vi "AWS Execute CMD.vi"(8 "error in (no error)":errorcluster, 11 "LV-Data.AWS CLI":refnum<class "LV-Data.AWS CLI.lvclass">) -> (0 "error out":errorcluster, 2 "std out":string, 3 "LV-Data.AWS CLI out":refnum<class "LV-Data.AWS CLI.lvclass">)   [LabVIEW 2019, in "LV-Data.AWS CLI.lvclass"]
uses:
  LV-Data.AWS CLI.lvclass
  <userlib>/_OpenG.lib/string/string.llb/Trim Whitespace (String)__ogtk.vi
panel:
  # "aws --version"
  # "aws s3 ls s3://levylab-data/CF900/"
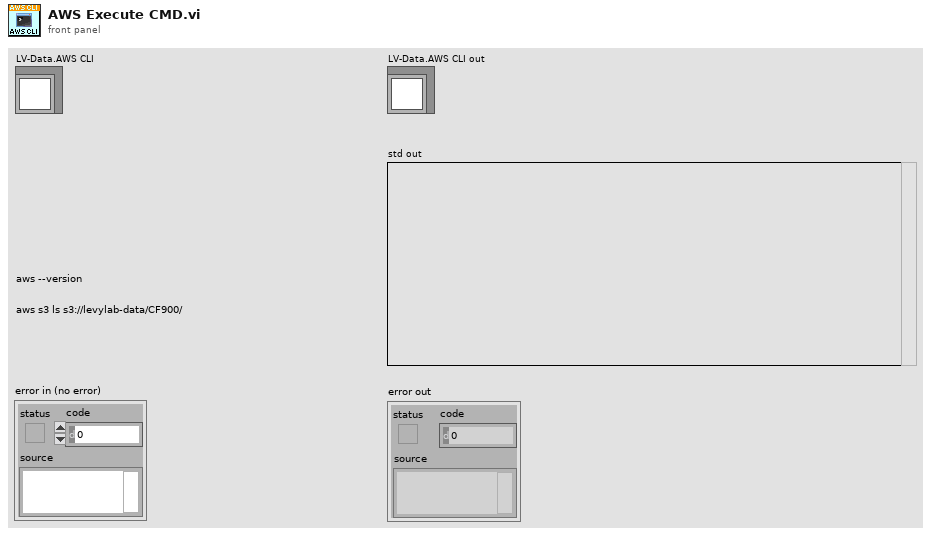
[diagram p1: front panel]
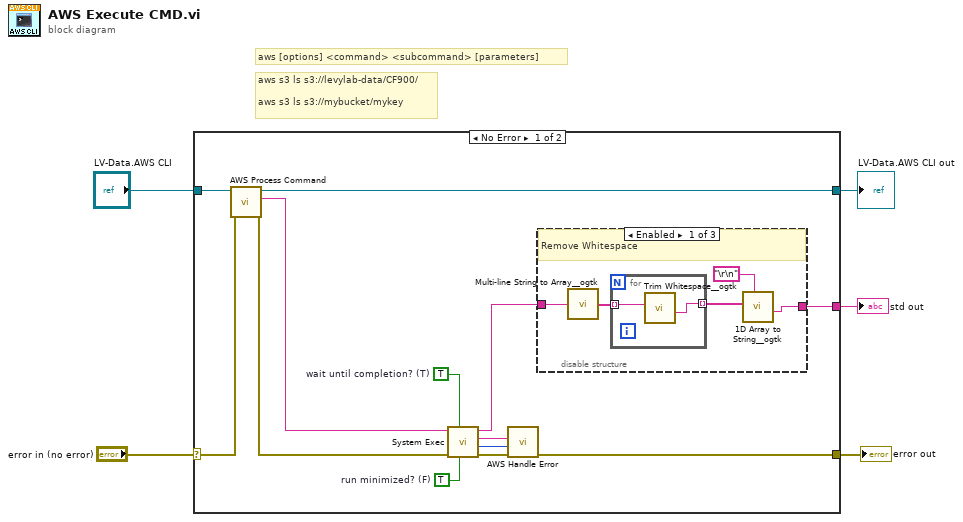
[diagram p0: block diagram]
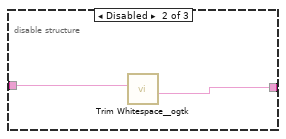
[diagram p2: hidden frame]
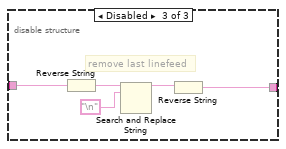
[diagram p3: hidden frame]
diagram:
  # "aws s3 ls s3://levylab-data/CF900/\n\naws s3 ls s3://mybucket/mykey"
  # "aws [options] <command> <subcommand> [parameters]"
  n1 = case shown="No Error" "error in (no error)" {
    selector: "error in (no error)" -> [w13 w34]
    tunnel: [w8 w34] -> w4
    tunnel: [w9 w33] -> w2
    tunnel: "LV-Data.AWS CLI" -> [w10 w33]
    tunnel: [w6 _] -> w1
    frame No Error {
      w17 = TRUE  # wait until completion? (T)
      w18 = TRUE  # run minimized? (F)
      n2 = call "AWS Process Command.vi"("error in"=w13, "LV-Data.AWS CLI"=w10) -> ("error out"=w12:errorcluster, "command line"=w11:string, "LV-Data.AWS CLI out"=w9:refnum<class "LV-Data.AWS CLI.lvclass">)  [unwired: 7 in]
      n3 = call <vilib>:"System Exec.vi"("run minimized? (F)"=w18, "wait until completion? (T)"=w17, "error in (no error)"=w12, "command line"=w11) -> ("error out"=w16:errorcluster, "return code"=w14:i32, "standard error"=w15:string, "standard output"=w7:string)  [unwired: 4 in]
      n4 = call "AWS Handle Error.vi"("error in (no error)"=w16, "return code"=w14, "standard error"=w15) -> ("error out"=w8:errorcluster)  [unwired: 8 in]
      n5 = disable-structure shown="Enabled" {
        disable-tunnel: w7 -> [w23 w27 w29]
        disable-tunnel: [w19 w26 w28] -> w6
        frame Enabled {
          # "Remove Whitespace"
          n6 = call <userlib>:"Multi-line String to Array__ogtk.vi"("string"=w23) -> ("lines"=w22:string[])
          n7 = for {
            tunnel: w22 -> [w25] mode=indexing
            tunnel: [w24] -> w20 mode=indexing
            n8 = call-poly <userlib>:"Trim Whitespace__ogtk.vi"("String in"=w25) -> ("String out"=w24:string)  [unwired: 6 in]
          }
          n9 = call <userlib>:"1D Array to String__ogtk.vi"("delimiter (Tab)"="\r\n", "Array of Strings"=w20) -> ("delimited string"=w19:string)  [unwired: 9 in]
        }
        frame Disabled {
          n10 = call-poly <userlib>:"Trim Whitespace__ogtk.vi"("String in"=w27) -> ("String out"=w26:string)  [unwired: 6 in]
        }
        frame Disabled {
          # "remove last linefeed"
          n11 = Reverse String(1:w29) -> (0:w32:string)
          n12 = Search and Replace String(input string=w32, search string="\n") -> (result string=w31:string)  [unwired: 6 in, 3 out]
          n13 = Reverse String(1:w31) -> (0:w28:string)
        }
      }
    }
    frame Error {
    }
  }
  "error out" <- w4
  "LV-Data.AWS CLI out" <- w2
  "std out" <- w1
